vi "Parse Full BB Topic Name.vi"(8 "error in":errorcluster, 11 "Full BB Topic Name":string) -> (0 "error out":errorcluster, 1 "Topic":string, 2 "Blackboard name":string, 3 "Plugin name":string)   [LabVIEW 2021, in "Iceoryx Channel Utilities.lvlib"]
uses:
  Iceoryx Channel Utilities.lvlib
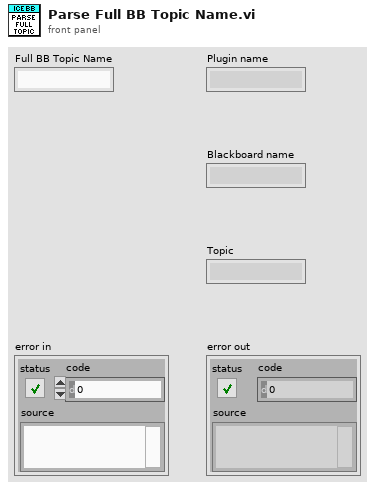
[diagram p1: front panel]
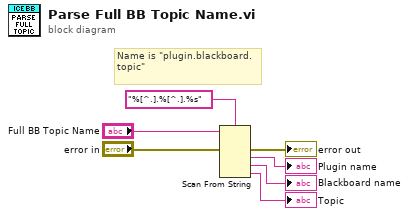
[diagram p0: block diagram]
diagram:
  # "Name is \"plugin.blackboard.topic\""
  n1 = Scan From String(format string="%[^.].%[^.].%s", input string="Full BB Topic Name", error in="error in") -> (error out=→"error out":errorcluster, output 1=→"Plugin name":string, output 2=→"Blackboard name":string, output 3=→"Topic":string)  [unwired: 4 in, 2 out]
